vi "Write U64 Direct.vi"(8 "error in (no error)":errorcluster, 10 "Data":u64, 11 "CIFTag in":refnum<class "CIF_Iceoryx_Chn_U64.lvclass">) -> (0 "error out":errorcluster, 3 "CIFTag out":refnum<class "CIF_Iceoryx_Chn_U64.lvclass">)   [LabVIEW 2021, in "CIF_Iceoryx_Chn_U64.lvclass"]
uses:
  CIF_Iceoryx_Chn_U64.lvclass
  D:/dev/Packages/CIF_Channels_Core/src/CIFChannels/CIFChannels.lvclass
  D:/dev/Packages/CIF_Channels_Core/src/Iceorxy_Channels/CIF_Iceoryx_BB/CIF_Iceoryx_BB.lvclass
  CIFChannels/CIFChannels.lvclass/CIFChannels.ctl
  CIF_Iceoryx_BB/CIF_Iceoryx_BB.lvclass/CIF_Iceoryx_BB.ctl
  CIF_Iceoryx_Chn_U64.lvclass/CIF_Iceoryx_Chn_U64.ctl
  CIFChannels/Accessors/Read Tag Forced.vi
  <vilib>/CIF Foundation/CIF Iceoryx/SubVIs/Get Path.vi
  <vilib>/CIF Foundation/CIF Iceoryx/SubVIs/Convert Error.vi
  <vilib>/CIF Foundation/CIF Iceoryx/Refnum/BB Writer from Refnum.vi
  <vilib>/CIF Foundation/CIF Iceoryx/SubVIs/Convert Error Core.vi
  0dfbf2d1-86f4-4cb3-9157-9e0b09da5a37.vi
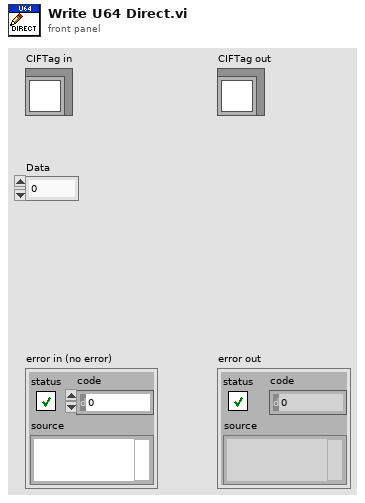
[diagram p1: front panel]
types:
  T1 = typedef "Iceoryx.lvlib/BB Writer Refnum.ctl" = cluster{"refnum":u64, "BB Writer":enum8{"bb_writer"}}
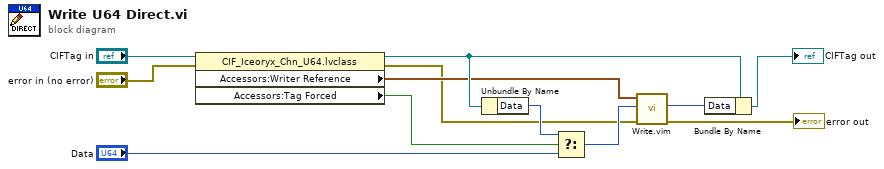
[diagram p0: block diagram]
diagram:
  n1 = property class="CIF_Iceoryx_Chn_U64.lvclass"(reference="CIFTag in", error in="error in (no error)") -> (reference out=w8:refnum<class "CIF_Iceoryx_Chn_U64.lvclass">, error out=w6:errorcluster, "Accessors:Writer Reference"=w7:T1, "Accessors:Tag Forced"=w9:bool)
  n2 = Unbundle By Name(w8) -> ("Data"=w12:u64)
  n3 = Select(t=w12, s=w9, f="Data") -> (s? t:f=w11:u64)
  n4 = call "Write.vim"("error in (no error)"=w6, "Data In"=w11, "Writer Reference"=w7) -> ("error out"=→"error out":errorcluster, "Data Out"=w10:u64)  [unwired: 7 in]
  n5 = Bundle By Name(cluster=w8, "Data"=w10) -> (→"CIFTag out":refnum<class "CIF_Iceoryx_Chn_U64.lvclass">)
